vi "包装工位查验.vi"(11 "客户码编号":string) -> (0 "长度":i32, 1 "干检OK":i32, 2 "氦检OK":i32, 3 "可否包装":bool, 4 "没氦检":bool, 5 "没包装码":bool, 6 "烘干工位号":string, 7 "已经烘干":bool, 8 "客户码数量":i32, 9 "上线码数量":i32, 10 "上线码":string)   [LabVIEW 2024]
panel:
  out "error out 2":errorcluster
  out "查重信息 2":string[][](array[string])
  out "长度 2":i32
  out "有客户码":bool
  out "结果字符串":string
  out "查重信息":string[][](array[string])
  out "error out":errorcluster
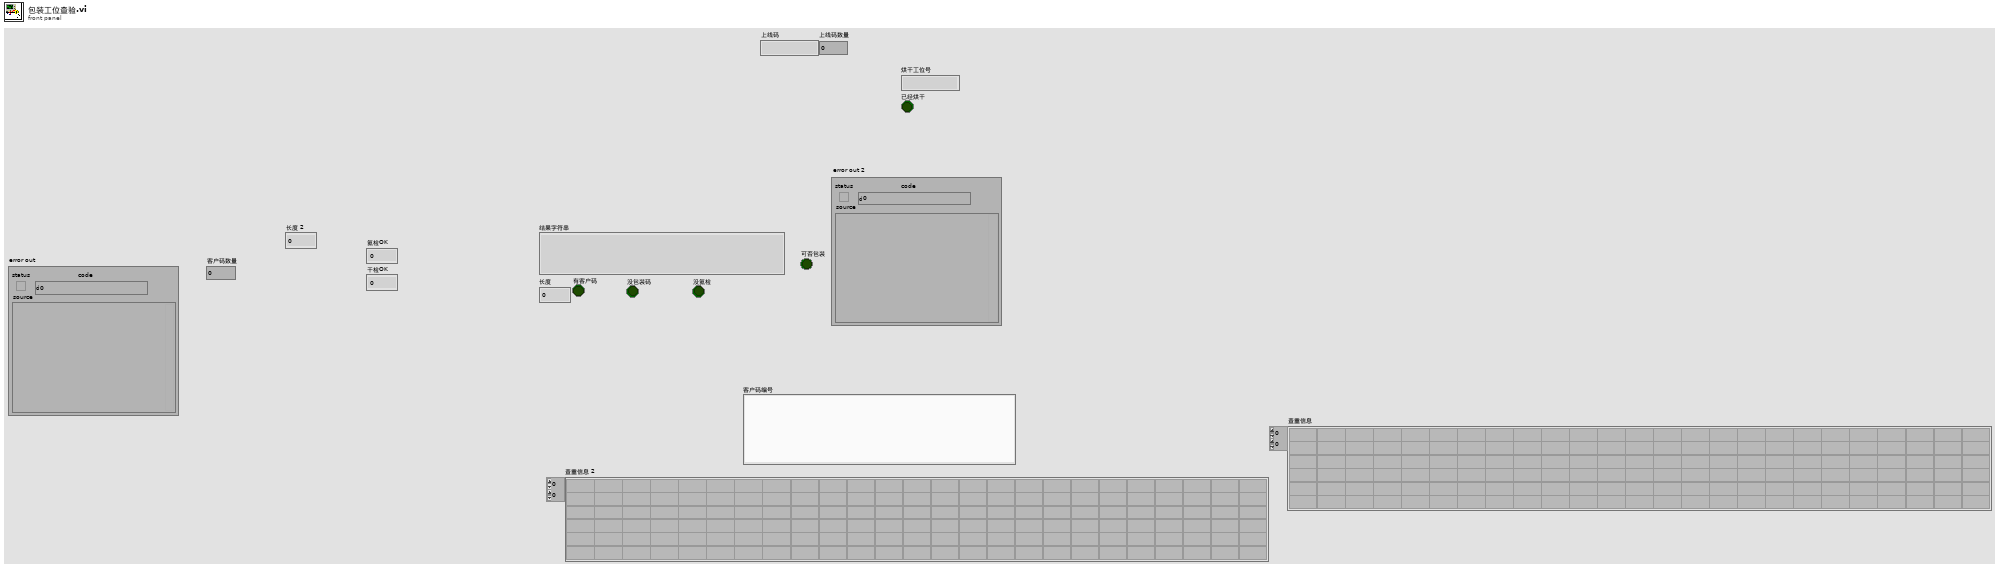
[diagram p1: front panel]
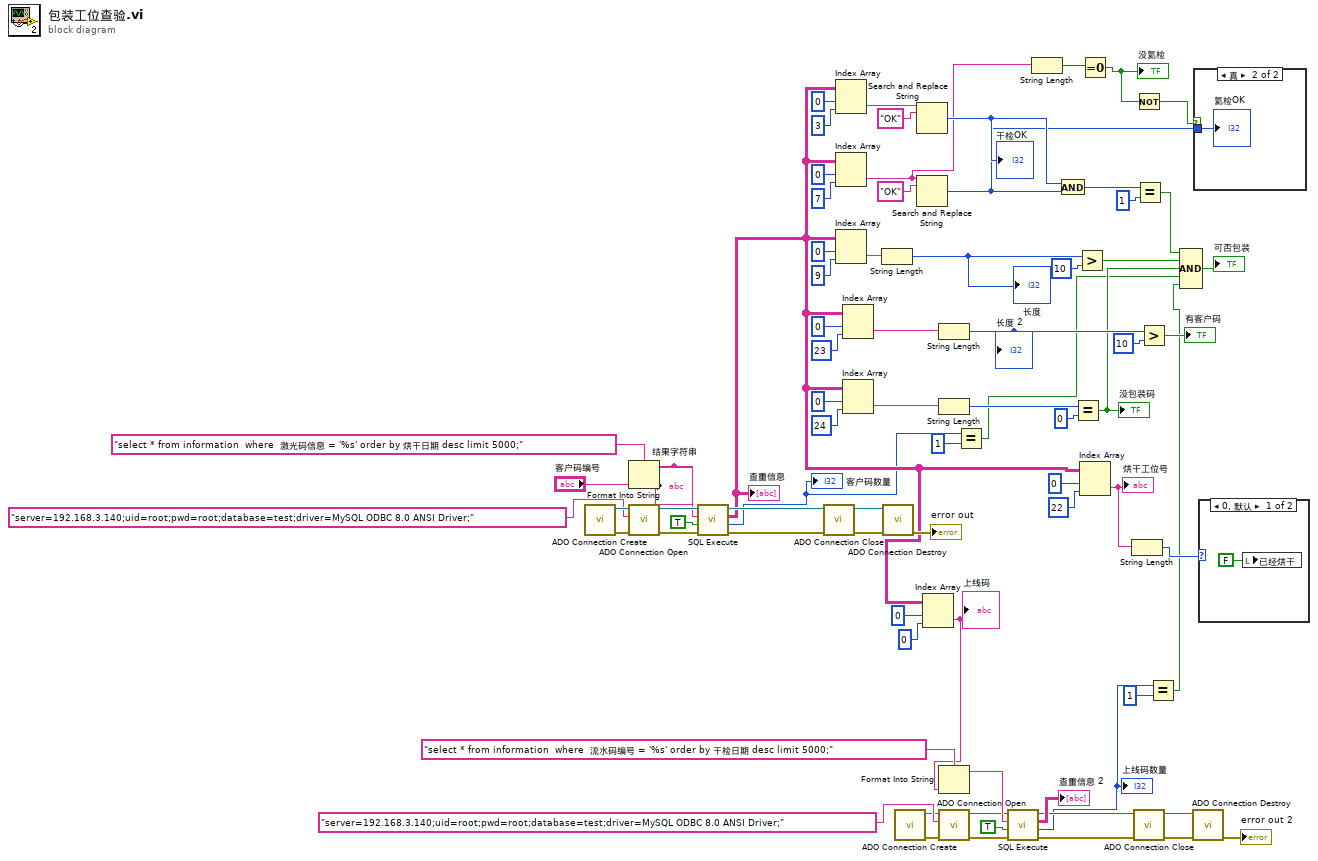
[diagram p0: block diagram]
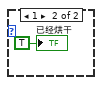
[diagram p2: hidden frame]
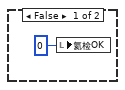
[diagram p3: hidden frame]
diagram:
  n1 = call "ADO Connection Create.vi"() -> ("error out"=w76:errorcluster, "ADODB._Connection Out"=w77:refnum<k7>)  [unwired: 10 in]
  n2 = Format Into String(format string="select * from information  where  激光码信息 = '%s' order by 烘干日期 desc limit 5000;" ("Command Text"), "客户码编号") -> (resulting string=w37:string)  [unwired: 2 in, 1 out]
  "结果字符串" <- w37
  n3 = call "ADO Connection Open.vi"("error in (no error)"=w76, "ConnectionString"="server=192.168.3.140;uid=root;pwd=root;database=test;driver=MySQL ODBC 8.0 ANSI Driver;", "ADODB._Connection In"=w77) -> ("error out"=w74:errorcluster, "ADODB._Connection Out"=w75:refnum<k7>)  [unwired: 7 in]
  n4 = call "SQL Execute.vi"("error in (no error)"=w74, "Return Data (T)"=TRUE, "Command Text"=w37, "ADODB._Connection In"=w75) -> ("error out"=w72:errorcluster, "Rows Fetched"=w2:i32, "Data"=w22:string[][], "ADODB._Connection Out"=w73:refnum<k7>)  [unwired: 4 in]
  "查重信息" <- w22
  "客户码数量" <- w2
  n5 = call "ADO Connection Close.vi"("error in (no error)"=w72, "ADODB._Connection In"=w73) -> ("error out"=w70:errorcluster, "ADODB._Connection Out"=w71:refnum<k7>)  [unwired: 8 in]
  n6 = Index Array(array=w22, index (row)=0 ("禁用的索引 (行)"), index (col)=3 ("禁用的索引 (列)")) -> (element=w61:string)
  n7 = Index Array(array=w22, index (row)=0 ("禁用的索引 (行)"), index (col)=7 ("禁用的索引 (列)")) -> (element=w32:string)
  n8 = Index Array(array=w22, index (row)=0 ("禁用的索引 (行)"), index (col)=9 ("禁用的索引 (列)")) -> (element=w55:string)
  n9 = Index Array(array=w22, index (row)=0 ("禁用的索引 (行)"), index (col)=23 ("禁用的索引 (列)")) -> (element=w49:string)
  n10 = Index Array(array=w22, index (row)=0 ("禁用的索引 (行)"), index (col)=24 ("禁用的索引 (列)")) -> (element=w44:string)
  n11 = String Length(string=w55) -> (length=w35:i32)
  "长度" <- w35
  n12 = call "ADO Connection Destroy.vi"("error in (no error)"=w70, "ADODB._Connection In"=w71) -> ("error out"=→"error out":errorcluster)  [unwired: 9 in]
  n13 = call "ADO Connection Create.vi"() -> ("error out"=w8:errorcluster, "ADODB._Connection Out"=w7:refnum<k7>)  [unwired: 10 in]
  n14 = Search and Replace String(input string=w61, search string="OK" ("搜索字符串")) -> (number of replacements=w59:i32)  [unwired: 6 in, 3 out]
  "干检OK" <- w59
  n15 = Search and Replace String(input string=w32, search string="OK" ("搜索字符串")) -> (number of replacements=w58:i32)  [unwired: 6 in, 3 out]
  n16 = Index Array(array=w22, index (row)=0 ("禁用的索引 (行)"), index (col)=0 ("禁用的索引 (列)")) -> (element=w6:string)
  "上线码" <- w6
  n17 = String Length(string=w49) -> (length=w50:i32)
  "长度 2" <- w50
  n18 = String Length(string=w44) -> (length=w43:i32)
  n19 = Format Into String(format string="select * from information  where  流水码编号 = '%s' order by 干检日期 desc limit 5000;" ("Command Text"), w6) -> (resulting string=w18:string)  [unwired: 2 in, 1 out]
  n20 = call "ADO Connection Open.vi"("error in (no error)"=w8, "ConnectionString"="server=192.168.3.140;uid=root;pwd=root;database=test;driver=MySQL ODBC 8.0 ANSI Driver;", "ADODB._Connection In"=w7) -> ("error out"=w10:errorcluster, "ADODB._Connection Out"=w9:refnum<k7>)  [unwired: 7 in]
  n21 = Equal?(x=w2, y=1) -> (x = y?=w1:bool)
  n22 = call "SQL Execute.vi"("error in (no error)"=w10, "Return Data (T)"=TRUE, "Command Text"=w18, "ADODB._Connection In"=w9) -> ("error out"=w12:errorcluster, "Rows Fetched"=w5:i32, "Data"=→"查重信息 2":string[][], "ADODB._Connection Out"=w11:refnum<k7>)  [unwired: 4 in]
  "上线码数量" <- w5
  n23 = String Length(string=w32) -> (length=w31:i32)
  n24 = And(x=w59, y=w58) -> (x .and. y?=w53:i32)
  n25 = Equal?(x=w43, y=0) -> (x = y?=w33:bool)
  "没包装码" <- w33
  n26 = Greater?(x=w35, y=10) -> (0:w40:bool)
  n27 = Equal To 0?(x=w31) -> (x = 0?=w30:bool)
  "没氦检" <- w30
  n28 = Index Array(array=w22, index (row)=0 ("禁用的索引 (行)"), index (col)=22 ("禁用的索引 (列)")) -> (element=w26:string)
  "烘干工位号" <- w26
  n29 = String Length(string=w26) -> (length=w25:i32)
  n30 = Not(x=w30) -> (.not. x?=w29:bool)
  n31 = call "ADO Connection Close.vi"("error in (no error)"=w12, "ADODB._Connection In"=w11) -> ("error out"=w14:errorcluster, "ADODB._Connection Out"=w13:refnum<k7>)  [unwired: 8 in]
  n32 = Equal?(x=w53, y=1) -> (x = y?=w41:bool)
  n33 = Greater?(x=w50, y=10) -> (0:→"有客户码":bool)
  n34 = Equal?(x=w5, y=1) -> (x = y?=w3:bool)
  n35 = Compound Arithmetic op=AND ("复合运算")(w41, w40, w33, w1, w3) -> (→"可否包装":bool)
  n36 = call "ADO Connection Destroy.vi"("error in (no error)"=w14, "ADODB._Connection In"=w13) -> ("error out"=→"error out 2":errorcluster)  [unwired: 9 in]
  n37 = case shown="真" w29 {
    tunnel: w58 -> [_ w79]
    frame False {
      n38 = local write "氦检OK"(0 ("氦检OK")) -> ()
    }
    frame True {
      "氦检OK" <- w79
    }
  }
  n39 = case shown="0, 默认" w25 {
    frame 0, Default {
      n40 = local write "已经烘干"(FALSE ("已经烘干")) -> ()
    }
    frame 1 {
      "已经烘干" <- TRUE ("已经烘干")
    }
  }
